vi "PanelController.vi"   [LabVIEW 2026]
uses:
  StateMachine/Globals.vi
types:
  T1 = typedef "System_State.ctl" = u16
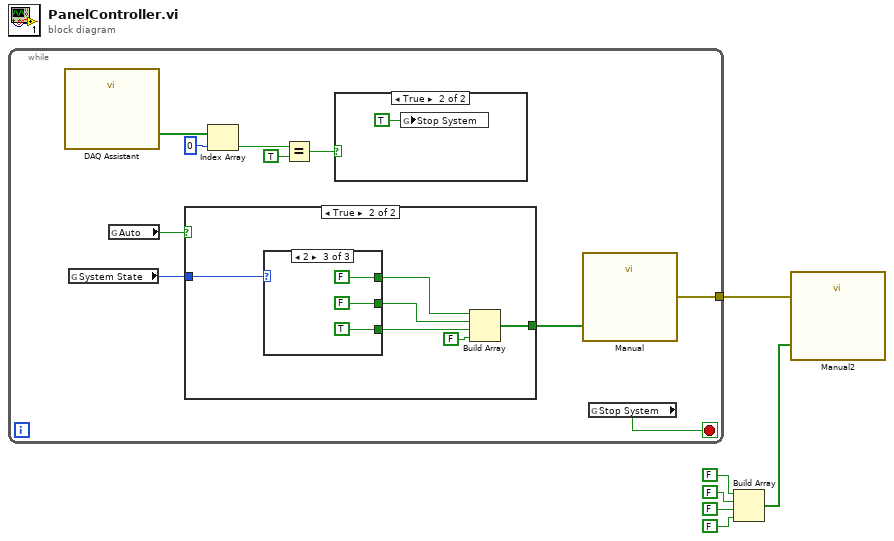
[diagram p0: block diagram]
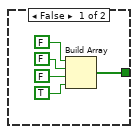
[diagram p3: hidden frame]
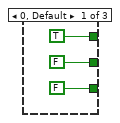
[diagram p4: hidden frame]
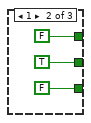
[diagram p5: hidden frame]
diagram:
  n1 = while {
    tunnel: [w11] -> w5
    stop <- w13 stop-if-true
    n2 = call "DAQ Assistant"() -> ("data"=w15:bool[])  [unwired: 17 in, 2 out]
    n3 = global read "Globals.vi" "System State"() -> (w10:T1)
    n4 = global read "Globals.vi" "Auto"() -> (w12:bool)
    n5 = case shown="True" w12 {
      tunnel: [w22 w24] -> w16
      tunnel: w10 -> [_ w28]
      frame False {
        n6 = Build Array(FALSE, FALSE, FALSE, TRUE) -> (w22:bool[])
      }
      frame True {
        n7 = case shown="2" w28 {
          tunnel: [TRUE FALSE FALSE] -> w27
          tunnel: [FALSE TRUE FALSE] -> w26
          tunnel: [FALSE FALSE TRUE] -> w25
          frame 0, Default {
          }
          frame 1 {
          }
          frame 2 {
          }
        }
        n8 = Build Array(w27, w26, w25, FALSE) -> (w24:bool[])
      }
    }
    n9 = Index Array(array=w15, index=0) -> (element=w9:bool)
    n10 = Equal?(x=w9, y=TRUE) -> (x = y?=w7:bool)
    n11 = case shown="True" w7 {
      frame False {
      }
      frame True {
        n12 = global write "Globals.vi" "Stop System"(TRUE ("Stop System")) -> ()
      }
    }
    n13 = call "Manual"("data"=w16) -> ("error out"=w11:errorcluster)  [unwired: 17 in, 1 out]
    n14 = global read "Globals.vi" "Stop System"() -> (w13:bool)
  }
  n15 = Build Array(FALSE, FALSE, FALSE, FALSE) -> (w6:bool[])
  n16 = call "Manual2"("data"=w6, "error in"=w5) -> ()  [unwired: 16 in, 2 out]
